vi "CSE Callback DlgDbg - Breakpoints & Colors.vi"(4 "Treat breakpoint":bool, 6 "Current Stm Line":i32=1, 7 "MCListbox Refnum":refnum<vi>, 8 "Line Number (1)":i32=1, 9 "Stm Idxs":i32[](array[numeric]), 10 "Line Nums":i32[](array[numeric]), 11 "CSE RefNum":T1) -> (0 "New Breakpoints":bool, 1 "Stm Idxs out":i32[](array[numeric]), 2 "Line Nums out":i32[](array[numeric]))   [LabVIEW 2021]
doc: "::: CalcExpress Toolkit :::\nCopyright (c) 2000-2026 Konstantin Shifershteyn. All rights reserved."
uses:
  vi.lib/addons/CalcExpress/cse.llb/CSE Instance RefNum.ctl
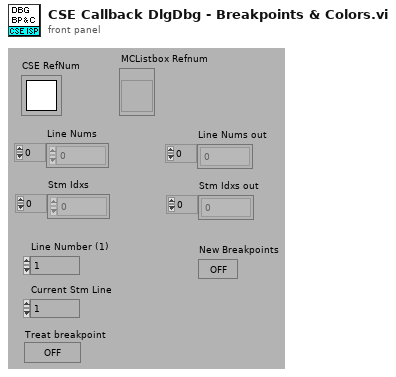
[diagram p1: front panel]
types:
  T1 = typedef "CSE Instance RefNum.ctl" = refnum<k1>
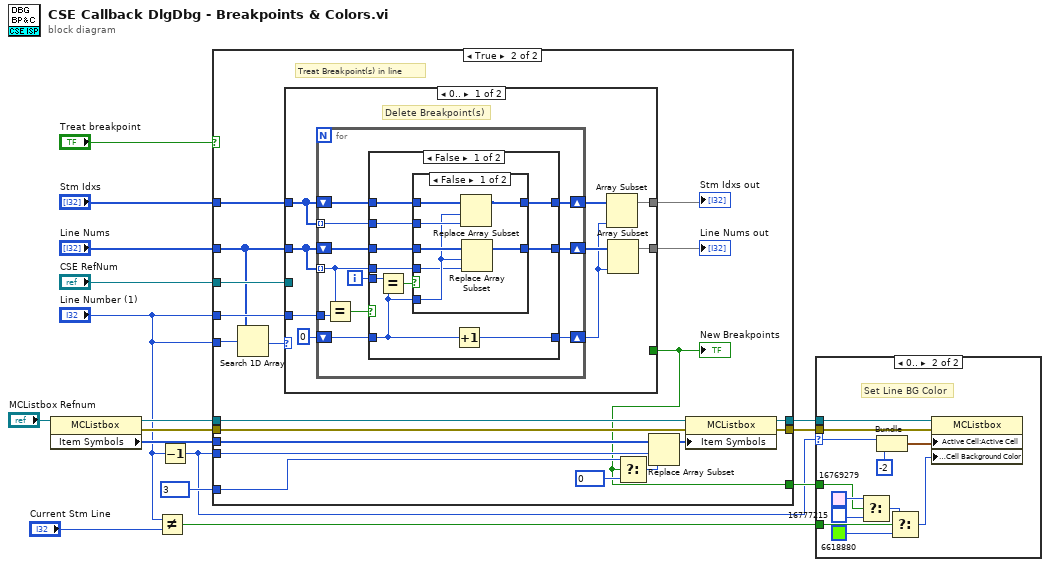
[diagram p0: block diagram]
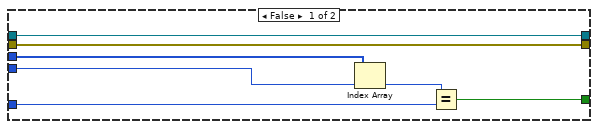
[diagram p3: hidden frame]
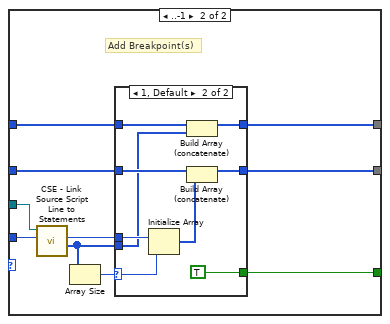
[diagram p6: hidden frame]
diagram:
  n1 = property class="MCListbox"(reference="MCListbox Refnum") -> (reference out=w11:refnum<vi>, error out=w10:errorcluster, "Item Symbols"=w12:i32[])  [unwired: 1 in]
  n2 = Not Equal?(x="Line Number (1)", y="Current Stm Line") -> (x != y?=w8:bool)
  n3 = Decrement(x="Line Number (1)") -> (x-1=w1:i32)
  n4 = case shown="True" "Treat breakpoint" {
    tunnel: "Line Number (1)" -> [_ w25]
    tunnel: "CSE RefNum" -> [_ w42]
    tunnel: "Line Nums" -> [_ w27]
    tunnel: "Stm Idxs" -> [_ w41]
    tunnel: w12 -> [w21 w36]
    tunnel: w11 -> [w23 w35]
    tunnel: w10 -> [w22 w34]
    tunnel: w1 -> [w20 w33]
    tunnel: "Line Number (1)" -> [_ w32]
    tunnel: [w23 w30] -> w7
    tunnel: [w22 w29] -> w6
    tunnel: 3 -> [w18 w28]
    tunnel: [w17 w24] -> w4
    frame False {
      n5 = Index Array(array=w21, index=w20) -> (element=w19:i32)
      n6 = Equal?(x=w19, y=w18) -> (x = y?=w17:bool)
    }
    frame True {
      # "Treat Breakpoint(s) in line"
      n7 = Search 1D Array(1D array=w27, element=w25) -> (index of element=w26:i32)  [unwired: 1 in]
      n8 = case shown="0.." w26 {
        tunnel: w42 -> [_ w94]
        tunnel: w32 -> [w51 w93]
        tunnel: w27 -> [w48 w91]
        tunnel: [w43 w90] -> w40
        tunnel: w41 -> [w49 w87]
        tunnel: [w44 w86] -> w39
        tunnel: [_ w85] -> w24
        frame 0.. {
          # "Delete Breakpoint(s)"
          n9 = for {
            shift-right: [w55] -> w47
            shift-left: w49 -> [w56]
            shift-right: [w57] -> w46
            shift-left: w48 -> [w58]
            tunnel: w51 -> [w62]
            shift-right: [w59] -> w45
            shift-left: 0 -> [w60]
            tunnel: w49 -> [w53] mode=indexing
            tunnel: w48 -> [w52] mode=indexing
            i -> [w54]
            n10 = Equal?(x=w52, y=w62) -> (x = y?=w61:bool)
            n11 = case shown="False" w61 {
              tunnel: w60 -> [w64 w84]
              tunnel: [w63 w84] -> w59
              tunnel: w58 -> [w69 w83]
              tunnel: [w68 w83] -> w57
              tunnel: w56 -> [w71 w82]
              tunnel: [w70 w82] -> w55
              tunnel: w54 -> [w72 _]
              tunnel: w53 -> [w67 _]
              tunnel: w52 -> [w66 _]
              frame False {
                n12 = Equal?(x=w72, y=w64) -> (x = y?=w65:bool)
                n13 = case shown="False" w65 {
                  tunnel: w71 -> [w79 w81]
                  tunnel: [w76 w81] -> w70
                  tunnel: w69 -> [w77 w80]
                  tunnel: [w75 w80] -> w68
                  tunnel: w64 -> [w74 _]
                  tunnel: w67 -> [w78 _]
                  tunnel: w66 -> [w73 _]
                  frame False {
                    n14 = Replace Array Subset(array=w79, new element=w78, index=w74) -> (w76:i32[])
                    n15 = Replace Array Subset(array=w77, new element=w73, index=w74) -> (w75:i32[])
                  }
                  frame True {
                  }
                }
                n16 = Increment(x=w64) -> (x+1=w63:i32)
              }
              frame True {
              }
            }
          }
          n17 = Array Subset(array=w47, length=w45) -> (w44:i32[])  [unwired: 1 in]
          n18 = Array Subset(array=w46, length=w45) -> (w43:i32[])  [unwired: 1 in]
        }
        frame ..-1 {
          # "Add Breakpoint(s)"
          n19 = call "CSE - Link Source Script Line to Statements.vi"("Line number (1)"=w93, "CSE RefNum"=w94) -> ("Stm Indexes"=w89:i32[], "dup Line number"=w88:i32)  [unwired: 6 in, 2 out]
          n20 = Array Size(array=w89) -> (size(s)=w92:i32)
          n21 = case shown="1, Default" w92 {
            selector: w92 -> [_ w105]
            tunnel: w91 -> [w96 w103]
            tunnel: [w96 w101] -> w90
            tunnel: w89 -> [_ w99]
            tunnel: w88 -> [_ w104]
            tunnel: w87 -> [w95 w100]
            tunnel: [w95 w98] -> w86
            tunnel: [_ TRUE] -> w85
            frame 0 {
            }
            frame 1, Default {
              n22 = Initialize Array(w104, w105) -> (w102:i32[])
              n23 = Build Array (concatenate)(w100, w99) -> (w98:i32[])
              n24 = Build Array (concatenate)(w103, w102) -> (w101:i32[])
            }
          }
        }
      }
      "Line Nums out" <- w40
      "Stm Idxs out" <- w39
      "New Breakpoints" <- w24
      n25 = Select(t=w28, s=w24, f=0) -> (s? t:f=w37:i32)
      n26 = Replace Array Subset(array=w36, new element=w37, index=w33) -> (w31:i32[])
      n27 = property class="MCListbox"(reference=w35, error in=w34, "Item Symbols"=w31) -> (reference out=w30:refnum<vi>, error out=w29:errorcluster)
    }
  }
  n28 = case shown="0.." w1 {
    selector: w1 -> [_ w106]
    tunnel: w8 -> [_ w115]
    tunnel: w7 -> [_ w111]
    tunnel: w6 -> [_ w110]
    tunnel: w4 -> [_ w108]
    frame ..-1 {
    }
    frame 0.. {
      # "Set Line BG Color"
      n29 = Select(t=u32 16769279, s=w108, f=u32 16777215) -> (s? t:f=w116:u32)
      n30 = Bundle(w106, -2) -> (w109:cluster{i32, i32})  [unwired: 1 in]
      n31 = Select(t=w116, s=w115, f=u32 6618880) -> (s? t:f=w107:u32)
      n32 = property class="MCListbox"(reference=w111, error in=w110, "Active Cell:Active Cell"=w109, "Active Cell:Cell Background Color"=w107) -> ()  [unwired: 2 out]
    }
  }
